vi "Watchdog Enable.vi"(4 "error in (no error)":errorcluster, 7 "watchdogID in":u64 format="%.0x") -> (0 "error out":errorcluster, 3 "watchdogID out":u64 format="%.0x")   [LabVIEW 2025]
doc: "<p>Enables the <a href=\"nihelplauncher://docs/csh?context=lvrt_lvrtconcepts_rt_watchdog\">watchdog object</a> and starts the countdown of the watchdog timer if the current status of the watchdog object is <strong>disabled</strong>.</p>"
uses:
  niwd4c.dll
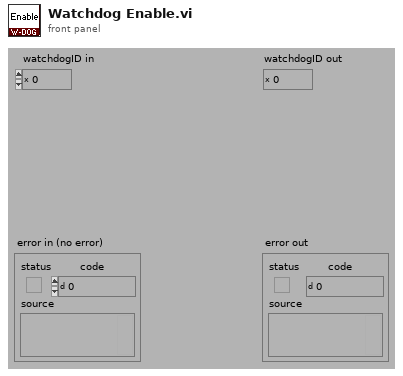
[diagram p1: front panel]
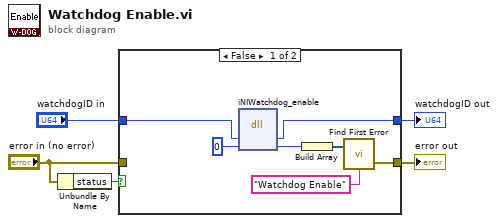
[diagram p0: block diagram]
diagram:
  n1 = Unbundle By Name("error in (no error)") -> ("status"=w5:bool)
  n2 = case shown="False" w5 {
    tunnel: [w8 w13] -> w1
    tunnel: [w11 w14] -> w2
    tunnel: "error in (no error)" -> [_ w14]
    tunnel: "watchdogID in" -> [w6 w13]
    frame False {
      n3 = dll-call lib="niwd4c.*" fn="iNIWatchdog_enable" label="Enable"("wd"=w6, "status"=0) -> ("wd"=w8:u64, "status"=w9:i32)  [unwired: 4 in, 2 out]
      n4 = Build Array(w9) -> (w12:i32[])
      n5 = call <vilib>:"Find First Error.vi"("source messages"="Watchdog Enable", "error codes"=w12) -> ("error out"=w11:errorcluster)  [unwired: 2 in, 1 out]
    }
    frame True {
    }
  }
  "error out" <- w2
  "watchdogID out" <- w1
